vi "serial.vi"() -> ()   [LabVIEW 2025]
uses:
  <vilib>/Instr/_visa.llb/VISA Configure Serial Port (Instr).vi
panel:
  out "read buffer":string
  in  "VISA resource name":refnum<visa-resource-name>
  in  "stop":bool
  out "Thermometer":dbl(slide) scale=0.0..100.0
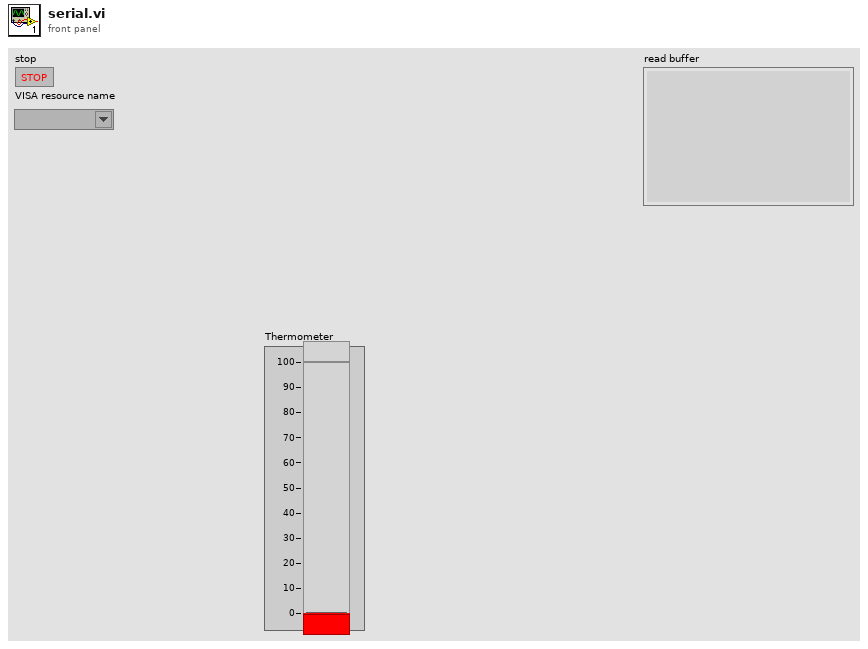
[diagram p1: front panel]
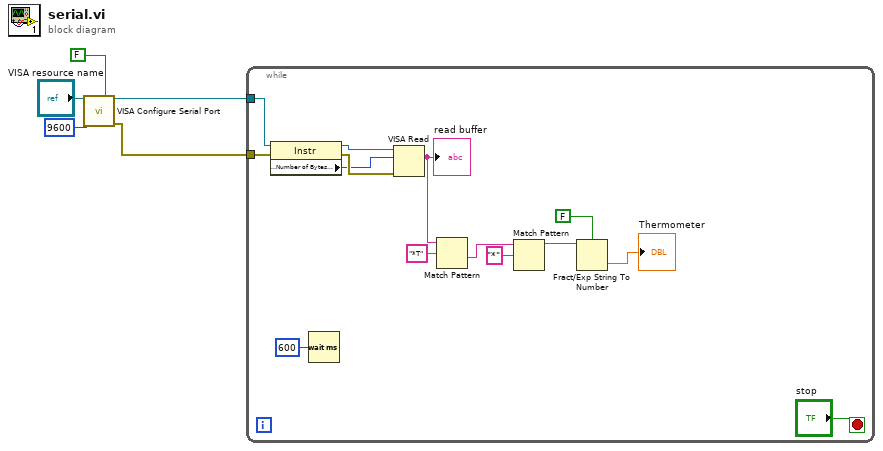
[diagram p0: block diagram]
diagram:
  n1 = call-poly "VISA Configure Serial Port"("VISA resource name"="VISA resource name", "Enable Termination\nChar (T)"=FALSE ("Enable Termination\nChar (T)"), "baud rate (9600)"=u32 9600) -> ("VISA resource name out"=w2:refnum<visa-resource-name>, "error out"=w1:errorcluster)  [unwired: 11 in]
  n2 = while {
    tunnel: w2 -> [w17]
    tunnel: w1 -> [w16]
    stop <- "stop" stop-if-true
    n3 = property class="Instr"(reference=w17, error in=w16) -> (reference out=w15:refnum<visa-resource-name>, error out=w14:errorcluster, "Serial Settings:Number of Bytes at Serial Port"=w13:u32)
    n4 = Wait (ms)(milliseconds to wait=u32 600) -> ()  [unwired: 1 out]
    n5 = VISA Read(VISA resource name=w15, byte count=w13, error in (no error)=w14) -> (read buffer=w12:string)  [unwired: 3 out]
    "read buffer" <- w12
    n6 = Match Pattern(string=w12, regular expression="*T") -> (after substring=w10:string)  [unwired: 1 in, 3 out]
    n7 = Match Pattern(string=w10, regular expression="*") -> (before substring=w8:string)  [unwired: 1 in, 3 out]
    n8 = Fract/Exp String To Number(use system decimal point (T)=FALSE, string=w8) -> (number=→"Thermometer":dbl)  [unwired: 2 in, 1 out]
  }
